vi "Test_DNL.vi"(0 "Values":refnum<vi>, 5 "Total":refnum<vi>, 11 "Error In":errorcluster) -> (4 "DNL":dbl[](array[numeric]), 6 "Codes Array":i32[](array[numeric]), 15 "Error Out":errorcluster)   [LabVIEW 2026, in "Core.lvlib"]
doc: "Calculates DNL values and updates result indicators using the supplied control references."
uses:
  Core.lvlib
  TypeDefs/Enum_Notifier_Name.ctl
  TypeDefs/Enum_Notifier_Options.ctl
  TypeDefs/Notification_Clusters/Cluster_DNL_Measurement_Specs.ctl
  <instrlib>/niDCPower/nidcpower.llb/niDCPower Output Function.ctl
  TypeDefs/Notification_Clusters/Cluster_ADC_Instrument_Specs.ctl
  TypeDefs/Notification_Clusters/Cluster_DAC_Instrument_Specs.ctl
  <instrlib>/niDCPower/nidcpower.llb/niDCPower Measurement Type.ctl
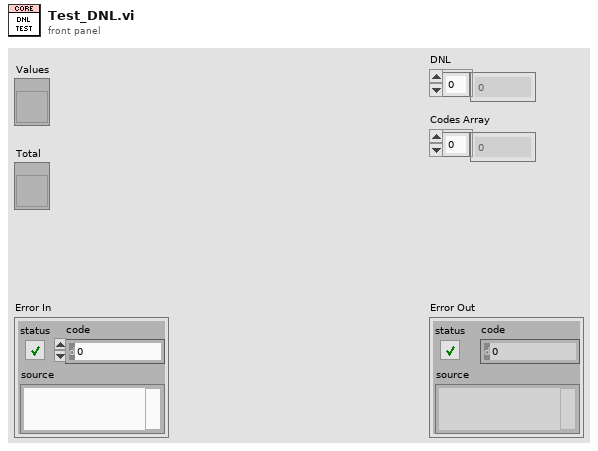
[diagram p1: front panel]
types:
  T1 = typedef "Core.lvlib/Cluster_DNL_Measurement_Specs.ctl" = cluster{" Resolution":u16, "Reference Voltage":dbl, "Settling Time (ms)":u32, "Start":dbl, "Step Size":dbl, "Stop":dbl}
  T2 = typedef "Core.lvlib/Enum_Notifier_Options.ctl" = enum16{"Create", "Send", "Status", "Release"}
  T3 = typedef "Core.lvlib/Enum_Notifier_Name.ctl" = enum16{"Device Type", "Test", "Instrument Spec", "Measurement Spec", "Status"}
  T4 = typedef "Core.lvlib/Cluster_ADC_Instrument_Specs.ctl" = cluster{"ADC Source":refnum<k15>, "Current Limit":dbl, "Voltage Level Range":dbl, "ADC DUT":string}
  T5 = typedef "Core.lvlib/Cluster_DAC_Instrument_Specs.ctl" = cluster{"DAC Measurement Device":refnum<k15>, "Current Limit":dbl, "Voltage Level Range":dbl, "DAC DUT":string}
  T6 = typedef "niDCPower Output Function.ctl" = i32
  T7 = typedef "niDCPower Measurement Type.ctl" = i32
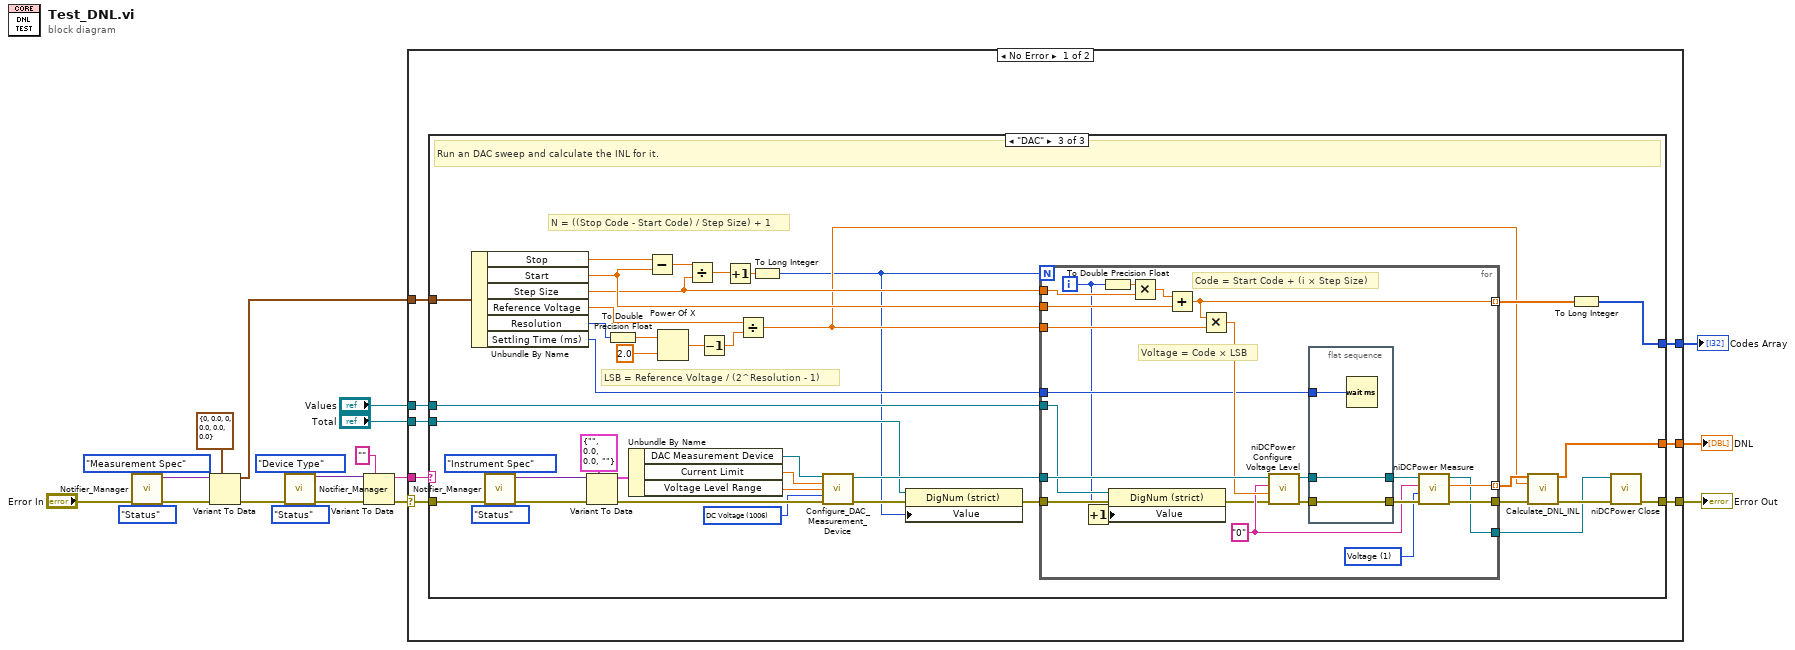
[diagram p0: block diagram]
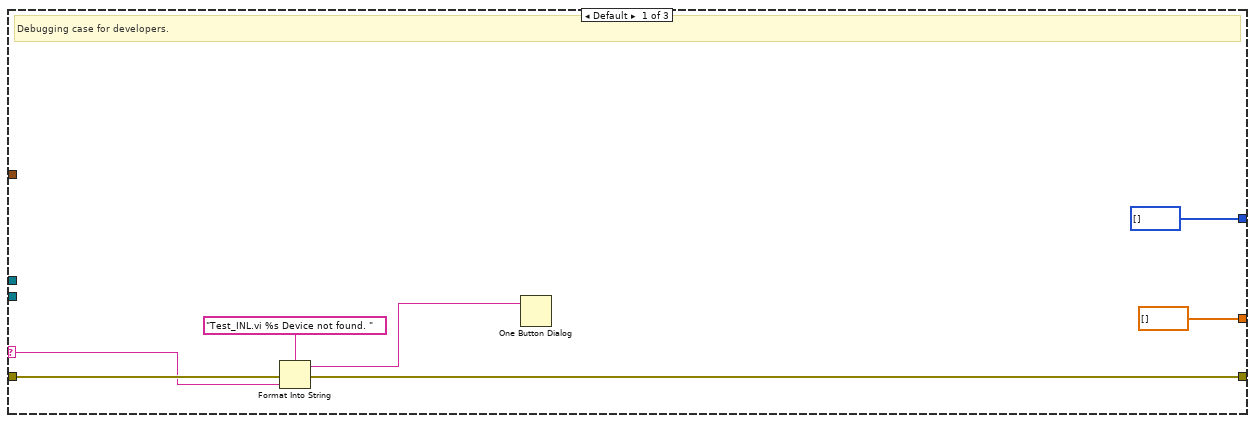
[diagram p2: hidden frame]
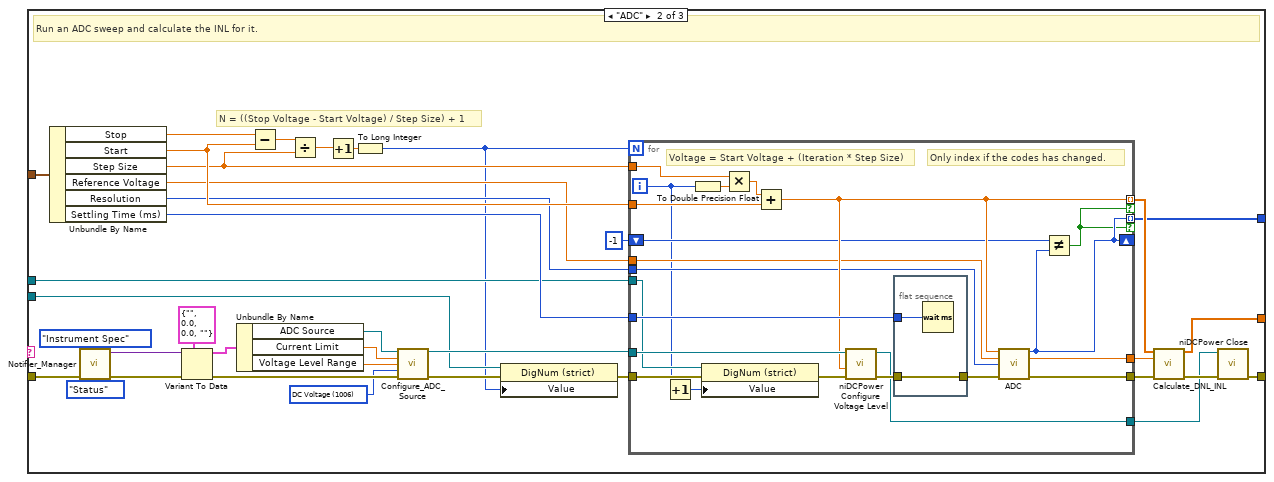
[diagram p3: hidden frame]
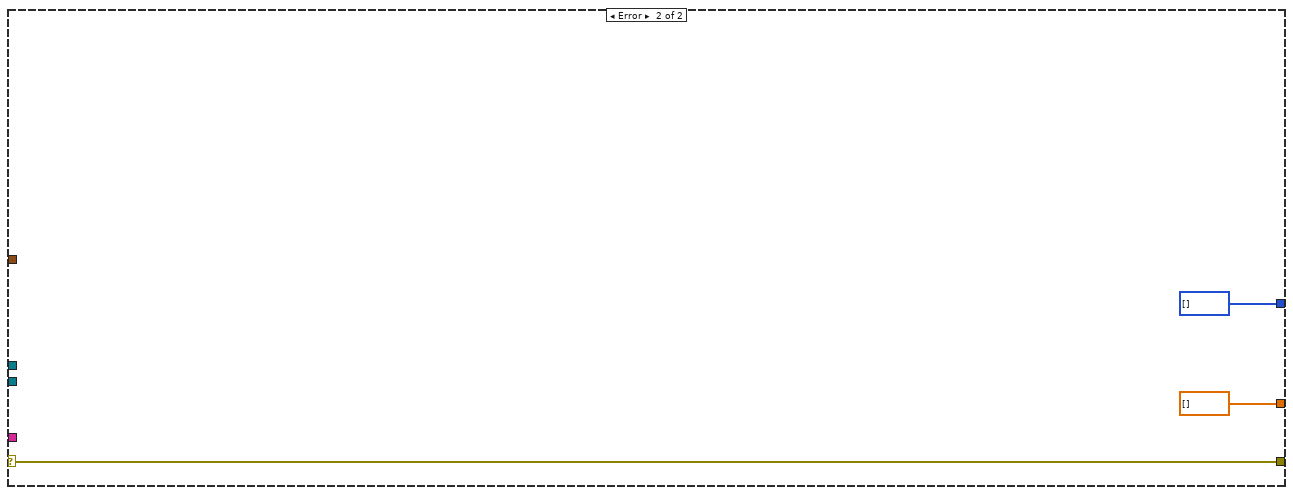
[diagram p4: hidden frame]
diagram:
  n1 = call "Notifier_Manager.vi"("Notifier Name"=Enum_Notifier_Name."Measurement Spec", "Error In"="Error In", "Notifier Options"=Enum_Notifier_Options."Status") -> ("Notifier Data"=w17:variant, "Error Out"=w15:errorcluster)  [unwired: 11 in]
  n2 = Variant To Data(error in=w15, type=T1 {" Resolution"=0, "Reference Voltage"=0.0, "Settling Time (ms)"=0, "Start"=0.0, "Step Size"=0.0, "Stop"=0.0} ("Measurement Specs"), Variant=w17) -> (data=w5:T1, error out=w16:errorcluster)
  n3 = call "Notifier_Manager.vi"("Notifier Name"=Enum_Notifier_Name."Device Type", "Error In"=w16, "Notifier Options"=Enum_Notifier_Options."Status") -> ("Notifier Data"=w14:variant, "Error Out"=w13:errorcluster)  [unwired: 11 in]
  n4 = Variant To Data(error in=w13, type="", Variant=w14) -> (data=w6:string, error out=w3:errorcluster)
  n5 = case shown="No Error" w3 {
    selector: w3 -> [w23 w166]
    tunnel: [w28 w166] -> w20
    tunnel: [w27 dbl[] [] ("INL")] -> w19
    tunnel: [w26 i32[] []] -> w18
    tunnel: w6 -> [w25 _]
    tunnel: w5 -> [w24 _]
    tunnel: "Values" -> [w22 _]
    tunnel: "Total" -> [w21 _]
    frame No Error {
      n6 = case shown="\"DAC\"" w25 {
        selector: w25 -> [w30 _ _]
        tunnel: w23 -> [w35 w70 w137]
        tunnel: [w32 w43 w105] -> w28
        tunnel: w24 -> [_ w53 w130]
        tunnel: [dbl[] [] ("INL") w41 w103] -> w27
        tunnel: [i32[] [] w45 w116] -> w26
        tunnel: w22 -> [_ w40 w102]
        tunnel: w21 -> [_ w38 w99]
        frame Default {
          # "Debugging case for developers."
          n7 = Format Into String(format string="Test_INL.vi %s Device not found. " ("message"), error in=w35, w30) -> (resulting string=w29:string, error out=w32:errorcluster)  [unwired: 1 in]
          n8 = One Button Dialog(message=w29) -> ()  [unwired: 1 in, 1 out]
        }
        frame "ADC" {
          w36 = T6 1006 items=["DC Voltage"=1006, "DC Current"=1007, "Pulse Voltage"=1049, "Pulse Current"=1050, "Constant Resistance"=1161, "Constant Power"=1162] ("output function")
          # "N = ((Stop Voltage - Start Voltage) / Step Size) + 1"
          # "Run an ADC sweep and calculate the INL for it."
          n9 = Unbundle By Name(w53) -> ("Stop"=w61:dbl, "Start"=w56:dbl, "Step Size"=w55:dbl, "Reference Voltage"=w51:dbl, "Resolution"=w50:u16, "Settling Time (ms)"=w52:u32)
          n10 = call "Notifier_Manager.vi"("Notifier Name"=Enum_Notifier_Name."Instrument Spec", "Error In"=w70, "Notifier Options"=Enum_Notifier_Options."Status") -> ("Notifier Data"=w65:variant, "Error Out"=w67:errorcluster)  [unwired: 11 in]
          n11 = Variant To Data(error in=w67, type=T4 {"ADC Source"="", "Current Limit"=0.0, "Voltage Level Range"=0.0, "ADC DUT"=""} ("ADC Instrument Spec"), Variant=w65) -> (data=w64:T4, error out=w63:errorcluster)
          n12 = Unbundle By Name(w64) -> ("ADC Source"=w62:refnum<k15>, "Current Limit"=w71:dbl, "Voltage Level Range"=w72:dbl)
          n13 = Subtract(x=w61, y=w56) -> (x-y=w60:dbl)
          n14 = Divide(x=w60, y=w55) -> (x/y=w59:dbl)
          n15 = Increment(x=w59) -> (x+1=w57:dbl)
          n16 = To Long Integer(number=w57) -> (32bit integer=w37:i32)
          n17 = call "Configure_ADC_Source.vi"("Resource Name"=w62, "Current Limit"=w71, "Voltage Level Range"=w72, "Output Function"=w36, "Error In"=w63) -> ("Instrument Handle"=w54:refnum<k15>, "Error Out"=w58:errorcluster)  [unwired: 9 in]
          n18 = property class="DigNum (strict)"(reference=w38, error in=w58, "Value"=w37) -> (error out=w39:errorcluster)  [unwired: 1 out]
          n19 = for {
            N: w37 -> [_]
            tunnel: w39 -> [w90]
            tunnel: w56 -> [w91]
            tunnel: w55 -> [w94]
            tunnel: [w85] -> w48 mode=indexing if=w77
            tunnel: w54 -> [w89]
            tunnel: w52 -> [w86]
            tunnel: w51 -> [w84]
            tunnel: w50 -> [w83]
            tunnel: [w82] -> w47
            tunnel: [w81] -> w42
            shift-right: [w78] -> _
            shift-left: -1 ("Code") -> [w80]
            tunnel: [w79] -> w46
            tunnel: [w78] -> w45 mode=indexing if=w77
            tunnel: w40 -> [w75]
            i -> [w74]
            # "Only index if the codes has changed."
            # "Voltage = Start Voltage + (Iteration * Step Size)"
            n20 = Increment(x=w74) -> (x+1=w73:i32)
            n21 = To Double Precision Float(number=w74) -> (double precision float=w93:dbl)
            n22 = property class="DigNum (strict)"(reference=w75, error in=w90, "Value"=w73) -> (error out=w76:errorcluster)  [unwired: 1 out]
            n23 = Multiply(x=w94, y=w93) -> (x*y=w92:dbl)
            n24 = Add(x=w92, y=w91) -> (x+y=w85:dbl)
            n25 = call <instrlib>:"niDCPower Configure Voltage Level.vi"("error in (no error)"=w76, "voltage level"=w85, "instrument handle"=w89) -> ("error out"=w88:errorcluster, "instrument handle out"=w81:refnum<k15>)  [unwired: 7 in]
            n26 = flat-sequence {
              tunnel: w88 -> [w96]
              tunnel: [w96] -> w87
              tunnel: w86 -> [w95]
              frame #0 {
                n27 = Wait (ms)(milliseconds to wait=w95) -> ()  [unwired: 1 out]
              }
            }
            n28 = call "ADC.vi"("Input Voltage"=w85, "Reference Voltage"=w84, "Resolution"=w83, "Error In"=w87) -> ("Code"=w78:i32, "LSB"=w79:dbl, "Error Out"=w82:errorcluster)  [unwired: 9 in]
            n29 = Not Equal?(x=w80, y=w78) -> (x != y?=w77:bool)
          }
          n30 = call "Calculate_DNL_INL.vi"("Transition Voltage"=w48, "LSB"=w46, "error in (no error)"=w47) -> ("DNL"=w41:dbl[], "error out"=w44:errorcluster)  [unwired: 10 in, 1 out]
          n31 = call <instrlib>:"niDCPower Close.vi"("error in (no error)"=w44, "instrument handle"=w42) -> ("error out"=w43:errorcluster)  [unwired: 9 in]
        }
        frame "DAC" {
          w97 = T6 1006 items=["DC Voltage"=1006, "DC Current"=1007, "Pulse Voltage"=1049, "Pulse Current"=1050, "Constant Resistance"=1161, "Constant Power"=1162] ("Output Function")
          # "N = ((Stop Code - Start Code) / Step Size) + 1"
          # "LSB = Reference Voltage / (2^Resolution - 1)"
          # "Run an DAC sweep and calculate the INL for it."
          n32 = Unbundle By Name(w130) -> ("Stop"=w120:dbl, "Start"=w119:dbl, "Step Size"=w118:dbl, "Reference Voltage"=w124:dbl, "Resolution"=w125:u16, "Settling Time (ms)"=w109:u32)
          n33 = call "Notifier_Manager.vi"("Notifier Name"=Enum_Notifier_Name."Instrument Spec", "Error In"=w137, "Notifier Options"=Enum_Notifier_Options."Status") -> ("Notifier Data"=w132:variant, "Error Out"=w134:errorcluster)  [unwired: 11 in]
          n34 = Variant To Data(error in=w134, type=T5 {"DAC Measurement Device"="", "Current Limit"=0.0, "Voltage Level Range"=0.0, "DAC DUT"=""} ("DAC Instrument Spec"), Variant=w132) -> (data=w131:T5, error out=w114:errorcluster)
          n35 = To Double Precision Float(number=w125) -> (double precision float=w128:dbl)
          n36 = Unbundle By Name(w131) -> ("DAC Measurement Device"=w113:refnum<k15>, "Current Limit"=w112:dbl, "Voltage Level Range"=w111:dbl)
          n37 = Subtract(x=w120, y=w119) -> (x-y=w123:dbl)
          n38 = Power Of X(1:2.0 ("x"), 2:w128) -> (0:w127:dbl)
          n39 = Divide(x=w123, y=w118) -> (x/y=w122:dbl)
          n40 = Decrement(x=w127) -> (x-1=w126:dbl)
          n41 = Increment(x=w122) -> (x+1=w121:dbl)
          n42 = Divide(x=w124, y=w126) -> (x/y=w107:dbl)
          n43 = To Long Integer(number=w121) -> (32bit integer=w98:i32)
          n44 = call "Configure_DAC_Measurement_Device.vi"("Measurement Device"=w113, "Current Limit"=w112, "Voltage Level Range"=w111, "Output Function"=w97, "Error In"=w114) -> ("Instrument Handle"=w110:refnum<k15>, "Error Out"=w100:errorcluster)  [unwired: 9 in]
          n45 = property class="DigNum (strict)"(reference=w99, error in=w100, "Value"=w98) -> (error out=w101:errorcluster)  [unwired: 1 out]
          n46 = for {
            N: w98 -> [_]
            tunnel: w119 -> [w157]
            tunnel: w118 -> [w160]
            tunnel: w107 -> [w156]
            tunnel: [w155] -> w117 mode=indexing
            tunnel: w101 -> [w154]
            tunnel: [w148] -> w115
            tunnel: w110 -> [w153]
            tunnel: w109 -> [w151]
            tunnel: [w144] -> w108 mode=indexing
            tunnel: [w143] -> w104
            tunnel: w102 -> [w140]
            i -> [w139]
            w142 = "0" ("channel name")
            w145 = T7 1 items=["Current", "Voltage"] ("measurement type")
            # "Voltage = Code × LSB"
            # "Code = Start Code + (i × Step Size)"
            n47 = Increment(x=w139) -> (x+1=w138:i32)
            n48 = To Double Precision Float(number=w139) -> (double precision float=w159:dbl)
            n49 = property class="DigNum (strict)"(reference=w140, error in=w154, "Value"=w138) -> (error out=w141:errorcluster)  [unwired: 1 out]
            n50 = Multiply(x=w159, y=w160) -> (x*y=w158:dbl)
            n51 = Add(x=w158, y=w157) -> (x+y=w155:dbl)
            n52 = Multiply(x=w155, y=w156) -> (x*y=w152:dbl)
            n53 = call <instrlib>:"niDCPower Configure Voltage Level.vi"("error in (no error)"=w141, "voltage level"=w152, "channel name"=w142, "instrument handle"=w153) -> ("error out"=w150:errorcluster, "instrument handle out"=w147:refnum<k15>)  [unwired: 6 in]
            n54 = flat-sequence {
              tunnel: w151 -> [w163]
              tunnel: w150 -> [w162]
              tunnel: [w162] -> w149
              tunnel: w147 -> [w161]
              tunnel: [w161] -> w146
              frame #0 {
                n55 = Wait (ms)(milliseconds to wait=w163) -> ()  [unwired: 1 out]
              }
            }
            n56 = call <instrlib>:"niDCPower Measure.vi"("error in (no error)"=w149, "measurement type"=w145, "channel name"=w142, "instrument handle"=w146) -> ("error out"=w148:errorcluster, "measurement"=w144:dbl, "instrument handle out"=w143:refnum<k15>)  [unwired: 5 in]
          }
          n57 = call "Calculate_DNL_INL.vi"("Transition Voltage"=w108, "LSB"=w107, "error in (no error)"=w115) -> ("DNL"=w103:dbl[], "error out"=w106:errorcluster)  [unwired: 10 in, 1 out]
          n58 = To Long Integer(number=w117) -> (32bit integer=w116:i32[])
          n59 = call <instrlib>:"niDCPower Close.vi"("error in (no error)"=w106, "instrument handle"=w104) -> ("error out"=w105:errorcluster)  [unwired: 9 in]
        }
      }
    }
    frame Error {
    }
  }
  "Error Out" <- w20
  "DNL" <- w19
  "Codes Array" <- w18
